vi "Measurement Logic.vi"() -> ()   [LabVIEW 2021, in "Crosstalk_PMIC.lvlib"]
uses:
  Crosstalk_PMIC.lvlib
  Measurement Configuration.ctl
  Measurement Results.ctl
  <vilib>/Plug-In SDKs/Measurements/Measure Call Context/Measure Call Context.lvclass
  <instrlib>/niDCPower/nidcpower.llb/niDCPower Sense.ctl
  <instrlib>/niDCPower/nidcpower.llb/niDCPower Source Mode.ctl
  <instrlib>/niDCPower/nidcpower.llb/niDCPower Wait For Event - Event.ctl
  <instrlib>/niDCPower/nidcpower.llb/niDCPower Measurement Type.ctl
  <instrlib>/niScope/Controls/niScope vertical coupling.ctl
  <instrlib>/niScope/Controls/niScope trigger slope.ctl
  <instrlib>/niScope/Controls/niScope trigger coupling.ctl
  <instrlib>/niScope/Controls/niScope trigger source.ctl
  <instrlib>/niDCPower/nidcpower.llb/niDCPower Get Channel Name From String.vi
  <instrlib>/niScope/Configure/Trigger/niScope Configure Trigger Edge.vi
  <instrlib>/niScope/Acquire/Fetch/niScope Multi Fetch WDT.vi
  <vilib>/Plug-In SDKs/Measurements/Measure Call Context/Accessor/Is Canceled.vi
panel:
  out "CrosstalkGraph":waveform(dbl)[](graph) caption="Ripple"
  out "measure call context out":refnum<class "Measure Call Context.lvclass">
  in  "measure call context in":refnum<class "Measure Call Context.lvclass">
  out "measurement results":T1
  in  "measurement configuration":T2={"Mode of operation"=enum."Perform measurement", "DUT setup time"=1.0, "Aperture time"=0.005, "Source resource name"="", "Source sense"=1009, "Source current limit"=25.0, "Source voltage level"=6.0, "Load resource name"="", "Load sense"=1009, "Load voltage limit range"=6.0, "Scope resource names"=[], "Scope channel names"=[], "Scope sample rate"=10000.0, "Scope acquisition time"=3.0, "Scope probe attenuation"=1.0, "Load current level"=0.005, "ExportData"=FALSE} {"Load sense" items=["Local"=1008, "Remote"=1009]; "Source sense" items=["Local"=1008, "Remote"=1009]}
  out "error out":errorcluster
  in  "error in":errorcluster
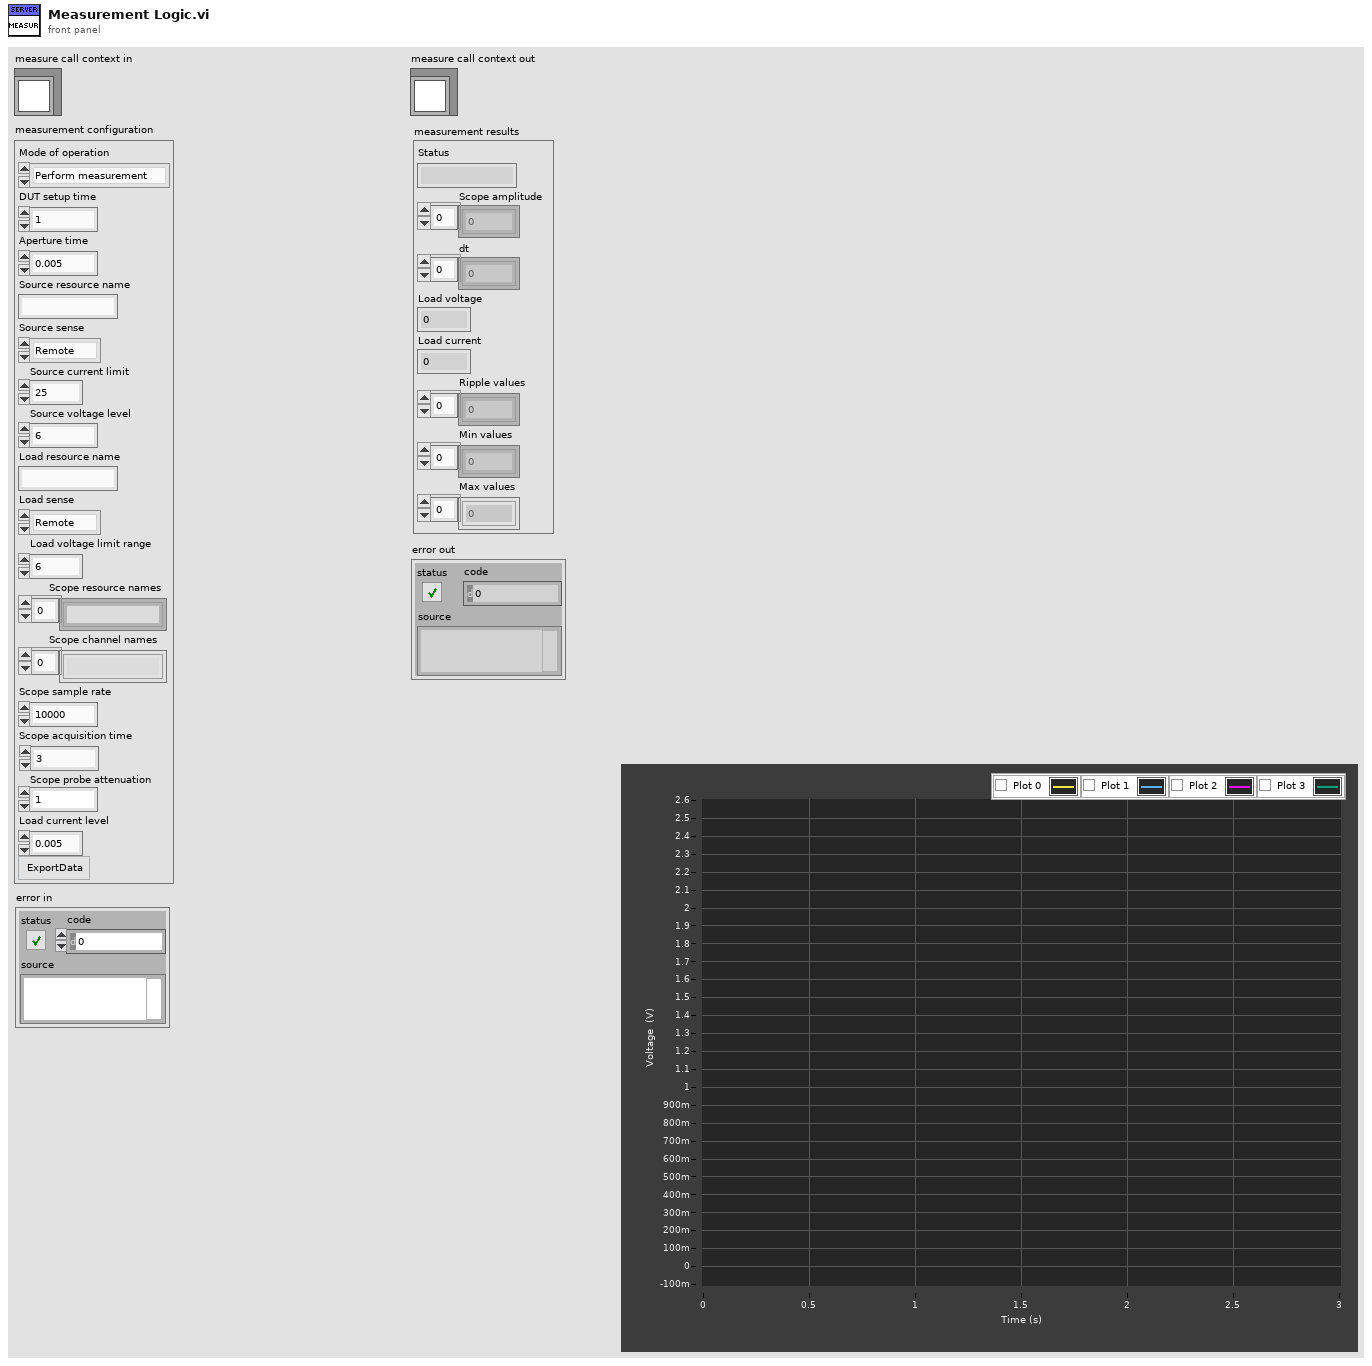
[diagram p1: front panel]
types:
  T1 = typedef "Crosstalk_PMIC.lvlib/Measurement Results.ctl" = cluster{"Status":string, "Scope amplitude":dbl[], "dt":dbl[], "Load voltage":dbl, "Load current":dbl, "Ripple values":dbl[], "Min values":dbl[], "Max values":dbl[]}
  T2 = typedef "Crosstalk_PMIC.lvlib/Measurement Configuration.ctl" = cluster{"Mode of operation":enum32{"Power on the DUT", "Perform measurement", "Power off the DUT"}, "DUT setup time":dbl, "Aperture time":dbl, "Source resource name":string, "Source sense":i32, "Source current limit":dbl, "Source voltage level":dbl, "Load resource name":string, "Load sense":i32, "Load voltage limit range":dbl, "Scope resource names":string[], "Scope channel names":string[], "Scope sample rate":dbl, "Scope acquisition time":dbl, "Scope probe attenuation":dbl, "Load current level":dbl, "ExportData":bool}
  T3 = cluster{"Source out":refnum<k15>, "Source channel name":string, "Load out":refnum<k15>, "Load channel name":string, "Scopes out":refnum<k15>[], "Scope channel names":string[], "Measurement Results":T1}
  T4 = enum32{"Power on the DUT", "Perform measurement", "Power off the DUT"}
  T5 = typedef "niScope trigger source.ctl" = string
  T6 = enum16{"open", "replace", "create", "open or create", "replace or create", "replace or create with confirmation"}
  T7 = typedef "niDCPower Wait For Event - Event.ctl" = i32
  T8 = typedef "niDCPower Source Mode.ctl" = i32
  T9 = typedef "niDCPower Sense.ctl" = i32
  T10 = typedef "niDCPower Measurement Type.ctl" = i32
  T11 = typedef "niScope vertical coupling.ctl" = i32
  T12 = typedef "niScope trigger coupling.ctl" = u16
  T13 = typedef "niScope trigger slope.ctl" = i32
  T14 = typedef "imagedata.ctl" = cluster{"image type":i32, "image depth":i32, "image":u8[], "mask":u8[], "colors":u32[], "Rectangle":cluster{"left":i16, "top":i16, "right":i16, "bottom":i16}}
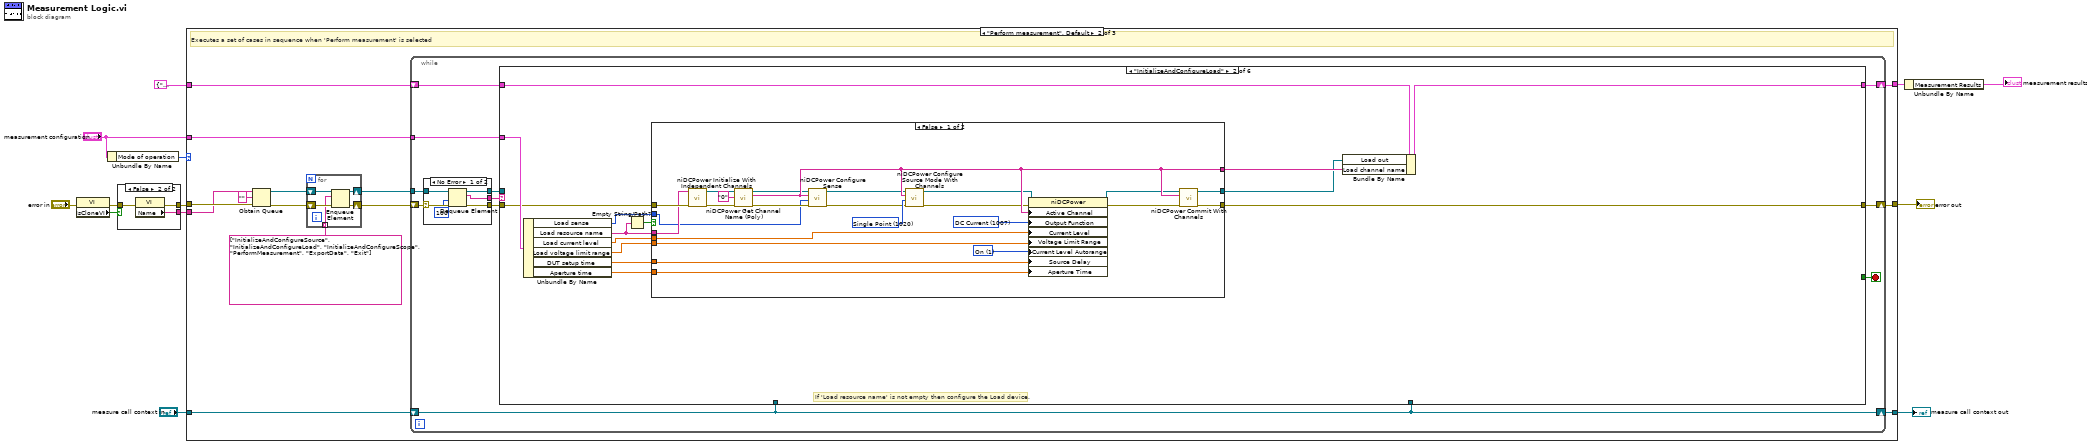
[diagram p0: block diagram]
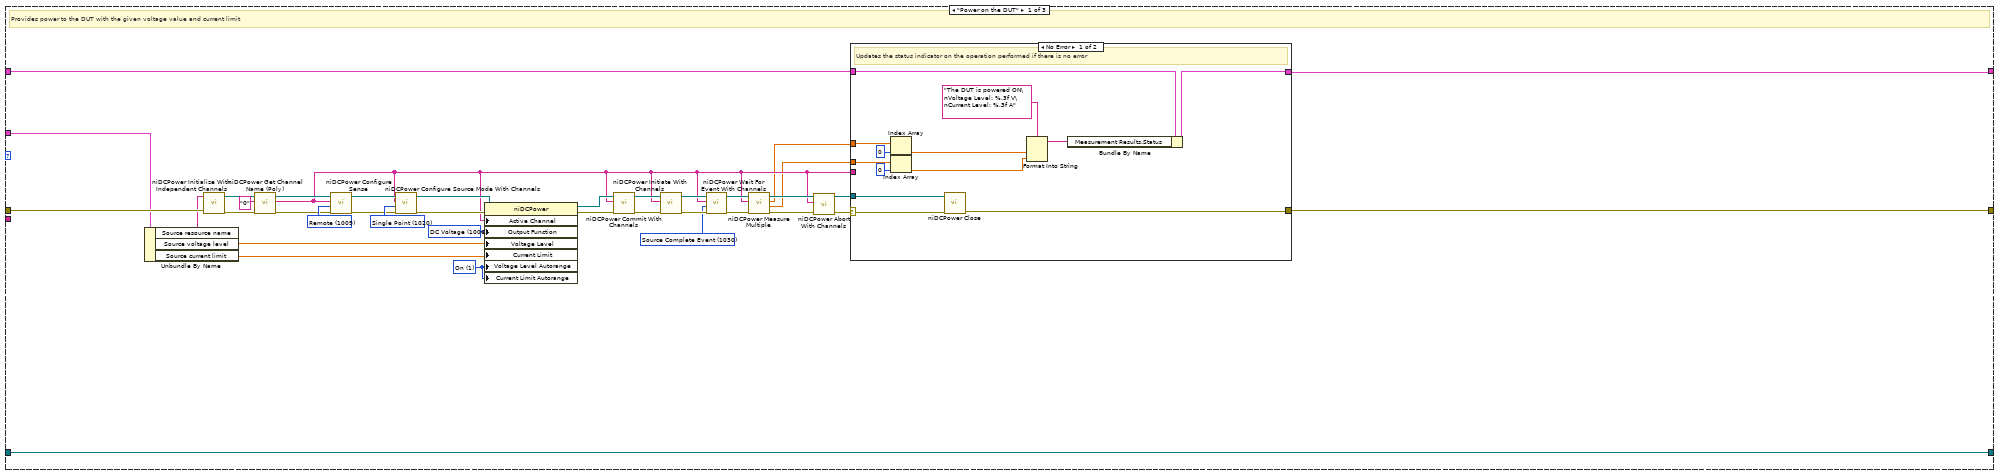
[diagram p2: hidden frame]
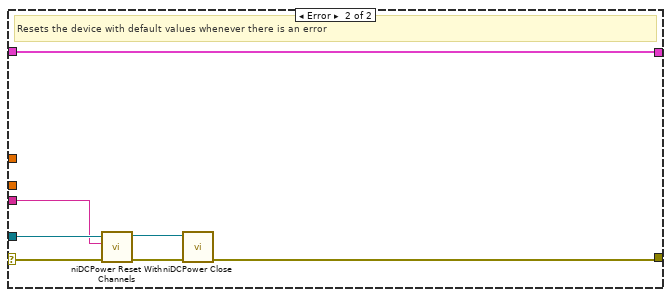
[diagram p3: hidden frame]
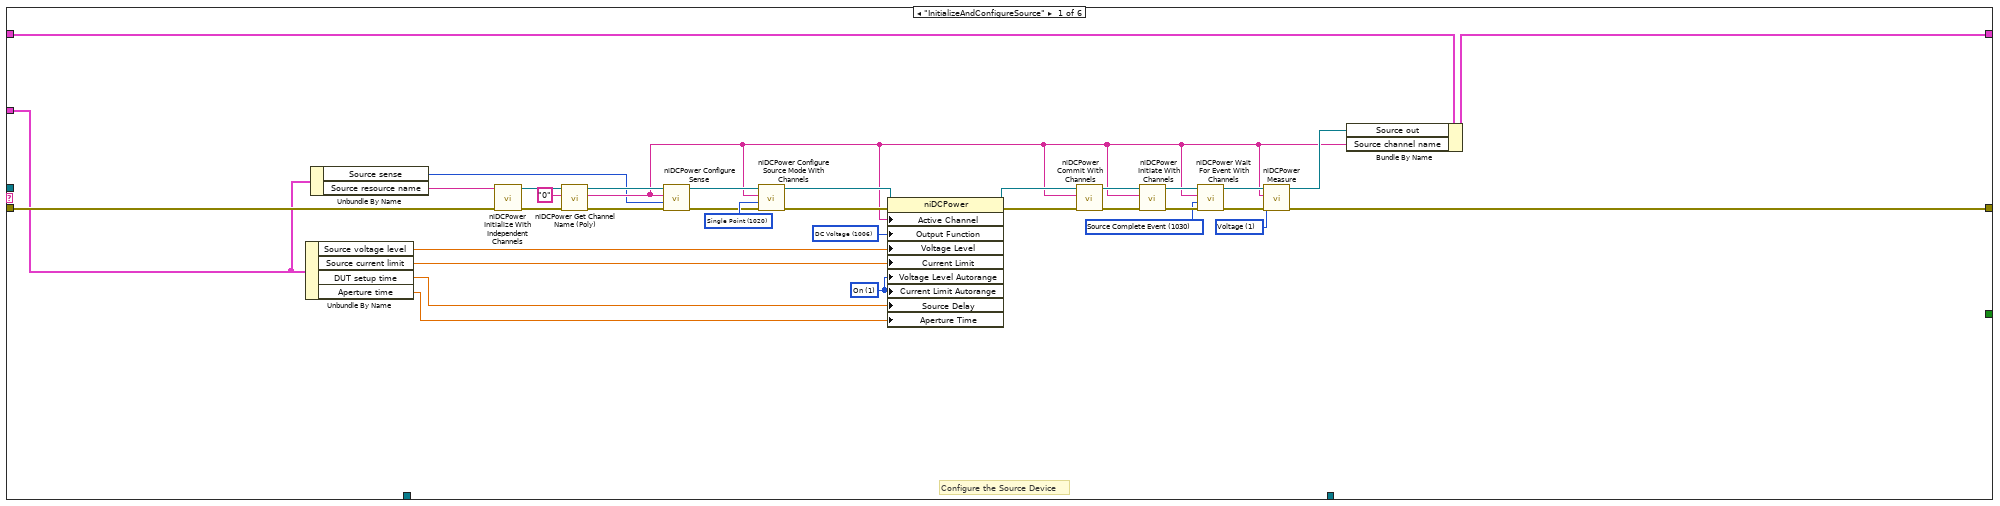
[diagram p4: hidden frame]
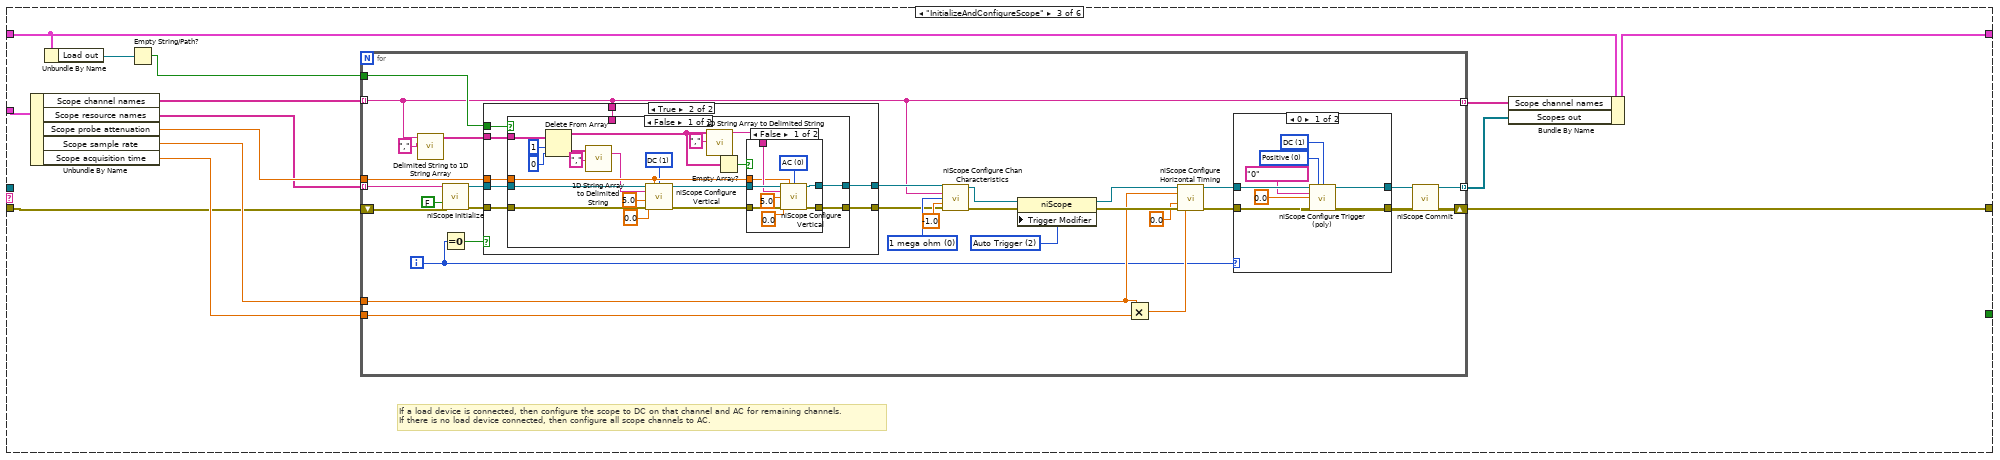
[diagram p6: hidden frame]
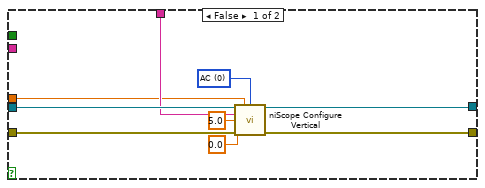
[diagram p7: hidden frame]
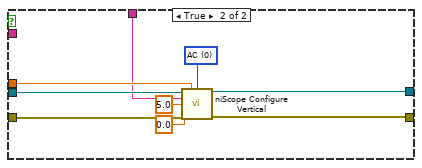
[diagram p9: hidden frame]
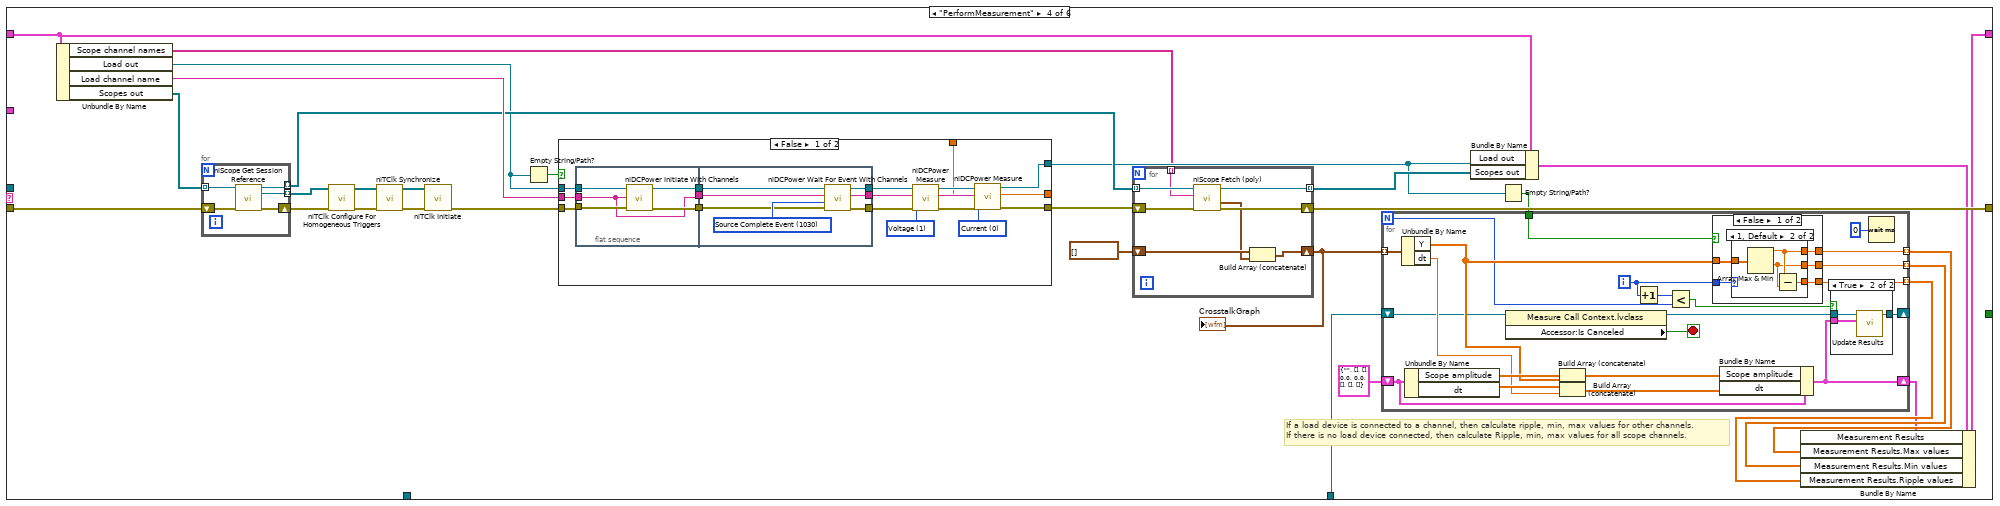
[diagram p11: hidden frame]
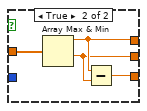
[diagram p15: hidden frame]
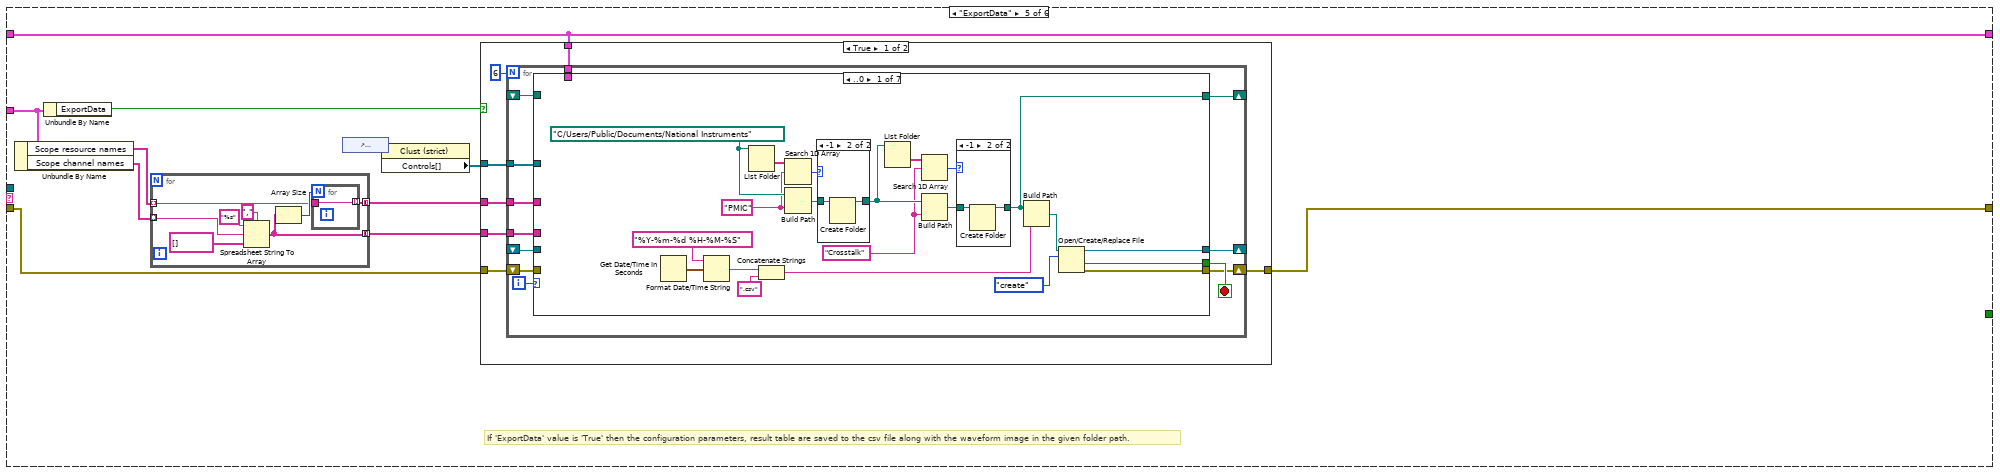
[diagram p16: hidden frame]
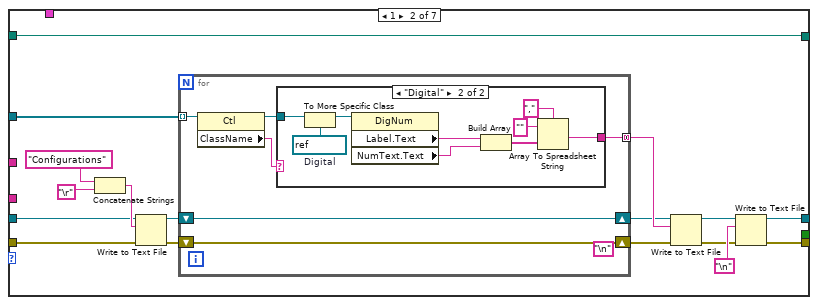
[diagram p19: hidden frame]
diagram:
  n1 = property class="VI"(error in="error in") -> (error out=w12:errorcluster, "IsCloneVI"=w13:bool)  [unwired: 1 in, 1 out]
  n2 = Unbundle By Name("measurement configuration") -> ("Mode of operation"=w7:T4)
  n3 = case shown="False" w13 {
    tunnel: [w16 w19] -> w10
    tunnel: [w15 w18] -> w9
    tunnel: w12 -> [w14 w17]
    frame True {
      n4 = property class="VI"(error in=w14) -> (error out=w16:errorcluster, "Clone Name"=w15:string)  [unwired: 1 in, 1 out]
    }
    frame False {
      n5 = property class="VI"(error in=w17) -> (error out=w19:errorcluster, "Name"=w18:string)  [unwired: 1 in, 1 out]
    }
  }
  n6 = case shown="\"Perform measurement\", Default" w7 {
    tunnel: [w21 w77 w667] -> w4
    tunnel: w10 -> [w37 w87 w666]
    tunnel: w9 -> [_ w86 _]
    tunnel: "measurement configuration" -> [w30 w83 w656]
    tunnel: [w22 w78 w653] -> w2
    tunnel: T3 {"Source out"="", "Source channel name"="", "Load out"="", "Load channel name"="", "Scopes out"=[], "Scope channel names"=[], "Measurement Results"={"Status"="", "Scope amplitude"=[], "dt"=[], "Load voltage"=0.0, "Load current"=0.0, "Ripple values"=[], "Min values"=[], "Max values"=[]}} -> [w23 w82 w654]
    tunnel: "measure call context in" -> [w20 w80 w655]
    tunnel: [w20 w79 w655] -> w5
    frame "Power on the DUT" {
      w40 = 1 items=["Off", "On"] ("Source:DC Voltage:Voltage Level Autorange")
      w41 = T7 1030 items=["Source Complete Event"=1030, "Measure Complete Event"=1031, "Sequence Iteration Complete Event"=1032, "Sequence Engine Done Event"=1033, "Pulse Complete Event"=1051, "Ready For Pulse Trigger Event"=1052] ("event")
      w52 = T8 1020 items=["Single Point"=1020, "Sequence"=1021] ("source mode")
      w47 = 1006 items=["DC Voltage"=1006, "DC Current"=1007, "Pulse Voltage"=1049, "Pulse Current"=1050] ("Source:Output Function")
      w42 = T9 1009 items=["Local"=1008, "Remote"=1009] ("sense")
      # "Provides power to the DUT with the given voltage value and current limit"
      n7 = Unbundle By Name(w30) -> ("Source resource name"=w34:string, "Source voltage level"=w29:dbl, "Source current limit"=w35:dbl)
      n8 = call <instrlib>:"niDCPower Initialize With Independent Channels.vi"("error in (no error)"=w37, "resource name"=w34) -> ("error out"=w39:errorcluster, "instrument handle out"=w43:refnum<k15>)  [unwired: 8 in]
      n9 = call-poly <instrlib>:"niDCPower Get Channel Name (Poly).vi"("index"="0", "instrument handle"=w43) -> ("name"=w26:string, "instrument handle out"=w38:refnum<k15>)  [unwired: 7 in, 1 out]
      n10 = call <instrlib>:"niDCPower Configure Sense.vi"("error in (no error)"=w39, "sense"=w42, "channel name"=w26, "instrument handle"=w38) -> ("error out"=w50:errorcluster, "instrument handle out"=w48:refnum<k15>)  [unwired: 6 in]
      n11 = call <instrlib>:"niDCPower Configure Source Mode With Channels.vi"("error in (no error)"=w50, "source mode"=w52, "channel name"=w26, "instrument handle"=w48) -> ("error out"=w51:errorcluster, "instrument handle out"=w49:refnum<k15>)  [unwired: 6 in]
      n12 = property class="niDCPower"(reference=w49, error in=w51, "Active Channel"=w26, "Output Function"=w47, "Voltage Level"=w29, "Current Limit"=w35, "Voltage Level Autorange"=w40, "Current Limit Autorange"=w40) -> (reference out=w53:refnum<k15>, error out=w54:errorcluster)
      n13 = call <instrlib>:"niDCPower Commit With Channels.vi"("error in (no error)"=w54, "channel name"=w26, "instrument handle"=w53) -> ("error out"=w56:errorcluster, "instrument handle out"=w55:refnum<k15>)  [unwired: 7 in]
      n14 = call <instrlib>:"niDCPower Initiate With Channels.vi"("error in (no error)"=w56, "channel name"=w26, "instrument handle"=w55) -> ("error out"=w44:errorcluster, "instrument handle out"=w45:refnum<k15>)  [unwired: 7 in]
      n15 = call <instrlib>:"niDCPower Wait For Event With Channels.vi"("error in (no error)"=w44, "event"=w41, "channel name"=w26, "instrument handle"=w45) -> ("error out"=w32:errorcluster, "instrument handle out"=w46:refnum<k15>)  [unwired: 6 in]
      n16 = call <instrlib>:"niDCPower Measure Multiple.vi"("error in (no error)"=w32, "channel name"=w26, "instrument handle"=w46) -> ("error out"=w31:errorcluster, "current measurements"=w24:dbl[], "voltage measurements"=w25:dbl[], "instrument handle out"=w33:refnum<k15>)  [unwired: 5 in]
      n17 = call <instrlib>:"niDCPower Abort With Channels.vi"("error in (no error)"=w31, "channel name"=w26, "instrument handle"=w33) -> ("error out"=w28:errorcluster, "instrument handle out"=w27:refnum<k15>)  [unwired: 7 in]
      n18 = case shown="No Error" w28 {
        selector: w28 -> [w69 w74]
        tunnel: [w68 w73] -> w21
        tunnel: [w67 w70] -> w22
        tunnel: w27 -> [w63 w72]
        tunnel: w26 -> [_ w71]
        tunnel: w25 -> [w62 _]
        tunnel: w24 -> [w61 _]
        tunnel: w23 -> [w60 w70]
        frame No Error {
          # "Updates the status indicator on the operation performed if there is no error"
          n19 = Index Array(array=w62, index=0) -> (element=w59:dbl)
          n20 = Index Array(array=w61, index=0) -> (element=w58:dbl)
          n21 = call <instrlib>:"niDCPower Close.vi"("error in (no error)"=w69, "instrument handle"=w63) -> ("error out"=w68:errorcluster)  [unwired: 9 out]
          n22 = Format Into String(format string="The DUT is powered ON\nVoltage Level: %.3f V\nCurrent Level: %.3f A" ("message"), w59, w58) -> (resulting string=w57:string)  [unwired: 2 in, 1 out]
          n23 = Bundle By Name(cluster=w60, "Measurement Results.Status"=w57) -> (w67:T3)
        }
        frame Error {
          # "Resets the device with default values whenever there is an error"
          n24 = call <instrlib>:"niDCPower Reset With Channels.vi"("error in (no error)"=w74, "channel name"=w71, "instrument handle"=w72) -> ("error out"=w76:errorcluster, "instrument handle out"=w75:refnum<k15>)  [unwired: 7 in]
          n25 = call <instrlib>:"niDCPower Close.vi"("error in (no error)"=w76, "instrument handle"=w75) -> ("error out"=w73:errorcluster)  [unwired: 9 out]
        }
      }
    }
    frame "Perform measurement", Default {
      # "Executes a set of cases in sequence when 'Perform measurement' is selected"
      n26 = Obtain Queue(name (unnamed)=w86, element data type="", error in (no error)=w87) -> (queue out=w89:refnum<queue>, error out=w90:errorcluster)  [unwired: 2 in, 1 out]
      n27 = for {
        shift-right: [w638] -> w84
        shift-left: w89 -> [w640]
        shift-right: [w637] -> w81
        shift-left: w90 -> [w639]
        tunnel: string[] ["InitializeAndConfigureSource", "InitializeAndConfigureLoad", "InitializeAndConfigureScope", "PerformMeasurement", "ExportData", "Exit"] ("Step sequence") -> [w636] mode=indexing
        n28 = Enqueue Element(queue=w640, element=w636, error in (no error)=w639) -> (queue out=w638:refnum<queue>, error out=w637:errorcluster)  [unwired: 1 in, 1 out]
      }
      n29 = while {
        tunnel: w84 -> [w101]
        tunnel: w83 -> [w98]
        shift-right: [w95] -> w78
        shift-left: w82 -> [w96]
        shift-right: [w94] -> w77
        shift-left: w81 -> [w100]
        shift-right: [w91] -> w79
        shift-left: w80 -> [w91]
        stop <- w93 stop-if-true
        n30 = case shown="No Error" w100 {
          selector: w100 -> [w630 w634]
          tunnel: w101 -> [w632 w633]
          tunnel: [w631 "Exit" ("t")] -> w92
          tunnel: [w629 w634] -> w97
          tunnel: [w627 w633] -> w99
          frame No Error {
            n31 = Dequeue Element(queue=w632, timeout in ms (-1)=100, error in (no error)=w630) -> (queue out=w627:refnum<queue>, element=w631:string, error out=w629:errorcluster)  [unwired: 1 out]
          }
          frame Error {
          }
        }
        n32 = case shown="\"InitializeAndConfigureLoad\"" w92 {
          tunnel: w99 -> [_ _ _ _ _ w569]
          tunnel: w98 -> [w112 w150 w189 _ w406 _]
          tunnel: w97 -> [w114 w149 w183 w306 w408 w574]
          tunnel: w96 -> [w133 w145 w178 w316 w400 w572]
          tunnel: [w134 w147 w184 w310 w400 w570] -> w95
          tunnel: [w136 w148 w182 w314 w407 w571] -> w94
          tunnel: w91 -> [_ _ _ _ _ _]
          tunnel: [_ _ _ _ _ TRUE] -> w93
          tunnel: w91 -> [_ _ _ w289 _ _]
          frame "InitializeAndConfigureSource" {
            w103 = T10 1 items=["Current", "Voltage"] ("measurement type")
            w116 = 1 items=["Off", "On"] ("Source:DC Voltage:Voltage Level Autorange")
            w117 = T7 1030 items=["Source Complete Event"=1030, "Measure Complete Event"=1031, "Sequence Iteration Complete Event"=1032, "Sequence Engine Done Event"=1033, "Pulse Complete Event"=1051, "Ready For Pulse Trigger Event"=1052] ("event")
            w128 = T8 1020 items=["Single Point"=1020, "Sequence"=1021] ("source mode")
            w123 = 1006 items=["DC Voltage"=1006, "DC Current"=1007, "Pulse Voltage"=1049, "Pulse Current"=1050] ("Source:Output Function")
            # "Configure the Source Device"
            n33 = Unbundle By Name(w112) -> ("Source voltage level"=w105:dbl, "Source current limit"=w113:dbl, "DUT setup time"=w115:dbl, "Aperture time"=w104:dbl)
            n34 = Unbundle By Name(w112) -> ("Source sense"=w102:i32, "Source resource name"=w111:string)
            n35 = call <instrlib>:"niDCPower Initialize With Independent Channels.vi"("error in (no error)"=w114, "resource name"=w111) -> ("error out"=w107:errorcluster, "instrument handle out"=w118:refnum<k15>)  [unwired: 8 in]
            n36 = call-poly <instrlib>:"niDCPower Get Channel Name (Poly).vi"("error in (no error)"=w107, "index"="0", "instrument handle"=w118) -> ("error out"=w106:errorcluster, "name"=w108:string, "instrument handle out"=w110:refnum<k15>)  [unwired: 6 in]
            n37 = call <instrlib>:"niDCPower Configure Sense.vi"("error in (no error)"=w106, "sense"=w102, "channel name"=w108, "instrument handle"=w110) -> ("error out"=w126:errorcluster, "instrument handle out"=w124:refnum<k15>)  [unwired: 6 in]
            n38 = call <instrlib>:"niDCPower Configure Source Mode With Channels.vi"("error in (no error)"=w126, "source mode"=w128, "channel name"=w108, "instrument handle"=w124) -> ("error out"=w127:errorcluster, "instrument handle out"=w125:refnum<k15>)  [unwired: 6 in]
            n39 = property class="niDCPower"(reference=w125, error in=w127, "Active Channel"=w108, "Output Function"=w123, "Voltage Level"=w105, "Current Limit"=w113, "Voltage Level Autorange"=w116, "Current Limit Autorange"=w116, "Source Delay"=w115, "Aperture Time"=w104) -> (reference out=w129:refnum<k15>, error out=w130:errorcluster)
            n40 = call <instrlib>:"niDCPower Commit With Channels.vi"("error in (no error)"=w130, "channel name"=w108, "instrument handle"=w129) -> ("error out"=w132:errorcluster, "instrument handle out"=w131:refnum<k15>)  [unwired: 7 in]
            n41 = call <instrlib>:"niDCPower Initiate With Channels.vi"("error in (no error)"=w132, "channel name"=w108, "instrument handle"=w131) -> ("error out"=w119:errorcluster, "instrument handle out"=w120:refnum<k15>)  [unwired: 7 in]
            n42 = call <instrlib>:"niDCPower Wait For Event With Channels.vi"("error in (no error)"=w119, "event"=w117, "channel name"=w108, "instrument handle"=w120) -> ("error out"=w122:errorcluster, "instrument handle out"=w121:refnum<k15>)  [unwired: 6 in]
            n43 = call <instrlib>:"niDCPower Measure.vi"("error in (no error)"=w122, "measurement type"=w103, "channel name"=w108, "instrument handle"=w121) -> ("error out"=w136:errorcluster, "instrument handle out"=w135:refnum<k15>)  [unwired: 5 in, 1 out]
            n44 = Bundle By Name(cluster=w133, "Source out"=w135, "Source channel name"=w108) -> (w134:T3)
          }
          frame "InitializeAndConfigureLoad" {
            # "If 'Load resource name' is not empty then configure the Load device."
            n45 = Unbundle By Name(w150) -> ("Load sense"=w137:i32, "Load resource name"=w139:string, "Load current level"=w141:dbl, "Load voltage limit range"=w142:dbl, "DUT setup time"=w146:dbl, "Aperture time"=w140:dbl)
            n46 = Empty String/Path?(string/path=w139) -> (empty?=w138:bool)
            n47 = case shown="False" w138 {
              tunnel: w149 -> [w174 w175]
              tunnel: [w173 w175] -> w148
              tunnel: w146 -> [w172 _]
              tunnel: [w171 _] -> w144
              tunnel: [w170 _] -> w143
              tunnel: w142 -> [w169 _]
              tunnel: w141 -> [w168 _]
              tunnel: w140 -> [w167 _]
              tunnel: w139 -> [w152 _]
              tunnel: w137 -> [w151 _]
              frame False {
                w164 = T8 1020 items=["Single Point"=1020, "Sequence"=1021] ("source mode")
                w157 = 1 items=["Off", "On"] ("Source:DC Current:Current Level Autorange")
                w158 = 1007 items=["DC Voltage"=1006, "DC Current"=1007, "Pulse Voltage"=1049, "Pulse Current"=1050] ("Source:Output Function")
                n48 = call <instrlib>:"niDCPower Initialize With Independent Channels.vi"("error in (no error)"=w174, "resource name"=w152) -> ("error out"=w154:errorcluster, "instrument handle out"=w159:refnum<k15>)  [unwired: 8 in]
                n49 = call-poly <instrlib>:"niDCPower Get Channel Name (Poly).vi"("error in (no error)"=w154, "index"="0", "instrument handle"=w159) -> ("error out"=w153:errorcluster, "name"=w171:string, "instrument handle out"=w156:refnum<k15>)  [unwired: 6 in]
                n50 = call <instrlib>:"niDCPower Configure Sense.vi"("error in (no error)"=w153, "sense"=w151, "channel name"=w171, "instrument handle"=w156) -> ("error out"=w161:errorcluster, "instrument handle out"=w160:refnum<k15>)  [unwired: 6 in]
                n51 = call <instrlib>:"niDCPower Configure Source Mode With Channels.vi"("error in (no error)"=w161, "source mode"=w164, "channel name"=w171, "instrument handle"=w160) -> ("error out"=w163:errorcluster, "instrument handle out"=w162:refnum<k15>)  [unwired: 6 in]
                n52 = property class="niDCPower"(reference=w162, error in=w163, "Active Channel"=w171, "Output Function"=w158, "Current Level"=w168, "Voltage Limit Range"=w169, "Current Level Autorange"=w157, "Source Delay"=w172, "Aperture Time"=w167) -> (reference out=w165:refnum<k15>, error out=w166:errorcluster)
                n53 = call <instrlib>:"niDCPower Commit With Channels.vi"("error in (no error)"=w166, "channel name"=w171, "instrument handle"=w165) -> ("error out"=w173:errorcluster, "instrument handle out"=w170:refnum<k15>)  [unwired: 7 in]
              }
              frame True {
              }
            }
            n54 = Bundle By Name(cluster=w145, "Load out"=w143, "Load channel name"=w144) -> (w147:T3)
          }
          frame "InitializeAndConfigureScope" {
            # "If a load device is connected, then configure the scope to DC on that channel and AC for remaining channels.\nIf there is no load device connected, then configure all scope channels to AC."
            n55 = Unbundle By Name(w189) -> ("Scope channel names"=w179:string[], "Scope resource names"=w180:string[], "Scope probe attenuation"=w188:dbl, "Scope sample rate"=w187:dbl, "Scope acquisition time"=w186:dbl)
            n56 = Unbundle By Name(w178) -> ("Load out"=w177:refnum<k15>)
            n57 = Empty String/Path?(string/path=w177) -> (empty?=w176:bool)
            n58 = for {
              tunnel: w180 -> [w207] mode=indexing
              tunnel: w179 -> [w192] mode=indexing
              tunnel: [w205] -> w185 mode=indexing
              tunnel: w188 -> [w194]
              tunnel: w187 -> [w204]
              tunnel: w186 -> [w203]
              shift-right: [w201] -> w182
              shift-left: w183 -> [w202]
              tunnel: [w192] -> w181 mode=indexing
              tunnel: w176 -> [w193]
              i -> [w191]
              w215 = 2 items=["None"=1, "Auto Trigger"=2] ("Triggering:Trigger Modifier")
              w219 = u32 0 items=["1 mega ohm"=0, "50 ohms"=2] ("input impedance")
              n59 = call <vilib>:"Delimited String to 1D String Array.vi"("delimiter"=",", "delimited string"=w192) -> ("string array"=w199:string[])  [unwired: 9 in]
              n60 = call <instrlib>:"niScope Initialize.vi"("resource name"=w207, "reset device"=FALSE, "error in"=w202) -> ("instrument handle"=w197:refnum<k15>, "error out"=w196:errorcluster)  [unwired: 11 in]
              n61 = Equal To 0?(x=w191) -> (x = 0?=w190:bool)
              n62 = case shown="True" w190 {
                tunnel: w199 -> [_ w237]
                tunnel: [w228 w236] -> w198
                tunnel: w197 -> [w229 w235]
                tunnel: w196 -> [w227 w234]
                tunnel: [w226 w233] -> w195
                tunnel: w194 -> [w221 w232]
                tunnel: w193 -> [_ w231]
                tunnel: w192 -> [w225 w230]
                frame False {
                  w224 = T11 0 items=["AC", "DC", "Ground"] ("vertical coupling")
                  n63 = call <instrlib>:"niScope Configure Vertical.vi"("instrument handle"=w229, "probe attenuation"=w221, "vertical coupling"=w224, "channels"=w225, "vertical range"=5.0, "vertical offset"=0.0, "error in"=w227) -> ("instrument handle out"=w228:refnum<k15>, "error out"=w226:errorcluster)  [unwired: 7 in]
                }
                frame True {
                  n64 = case shown="False" w231 {
                    tunnel: w237 -> [w257 _]
                    tunnel: [w253 w276] -> w236
                    tunnel: w235 -> [w252 w277]
                    tunnel: w234 -> [w251 w275]
                    tunnel: [w250 w274] -> w233
                    tunnel: w232 -> [w248 w270]
                    tunnel: w230 -> [_ w269]
                    frame False {
                      w243 = T11 1 items=["AC", "DC", "Ground"] ("vertical coupling")
                      n65 = Delete From Array(array=w257, length=1, index=0) -> (deleted portion=w246:string[], array with subset deleted=w238:string[])
                      n66 = call <vilib>:"1D String Array to Delimited String.vi"("delimiter"=",", "string array"=w246) -> ("delimited string"=w247:string)  [unwired: 9 in]
                      n67 = call <instrlib>:"niScope Configure Vertical.vi"("instrument handle"=w252, "probe attenuation"=w248, "vertical coupling"=w243, "channels"=w247, "vertical range"=5.0, "vertical offset"=0.0, "error in"=w251) -> ("instrument handle out"=w254:refnum<k15>, "error out"=w249:errorcluster)  [unwired: 7 in]
                      n68 = call <vilib>:"1D String Array to Delimited String.vi"("delimiter"=",", "string array"=w238) -> ("delimited string"=w239:string)  [unwired: 9 in]
                      n69 = Empty Array?(array=w238) -> (empty?=w240:bool)
                      n70 = case shown="False" w240 {
                        tunnel: w254 -> [w266 w268]
                        tunnel: w239 -> [w265 _]
                        tunnel: [w264 w268] -> w253
                        tunnel: [w263 w267] -> w250
                        tunnel: w249 -> [w262 w267]
                        tunnel: w248 -> [w258 _]
                        frame False {
                          w260 = T11 0 items=["AC", "DC", "Ground"] ("vertical coupling")
                          n71 = call <instrlib>:"niScope Configure Vertical.vi"("instrument handle"=w266, "probe attenuation"=w258, "vertical coupling"=w260, "channels"=w265, "vertical range"=5.0, "vertical offset"=0.0, "error in"=w262) -> ("instrument handle out"=w264:refnum<k15>, "error out"=w263:errorcluster)  [unwired: 7 in]
                        }
                        frame True {
                        }
                      }
                    }
                    frame True {
                      w271 = T11 0 items=["AC", "DC", "Ground"] ("vertical coupling")
                      n72 = call <instrlib>:"niScope Configure Vertical.vi"("instrument handle"=w277, "probe attenuation"=w270, "vertical coupling"=w271, "channels"=w269, "vertical range"=5.0, "vertical offset"=0.0, "error in"=w275) -> ("instrument handle out"=w276:refnum<k15>, "error out"=w274:errorcluster)  [unwired: 7 in]
                    }
                  }
                }
              }
              n73 = call <instrlib>:"niScope Configure Chan Characteristics.vi"("instrument handle"=w198, "channels"=w192, "input impedance"=w219, "maximum input frequency"=-1.0, "error in"=w195) -> ("instrument handle out"=w217:refnum<k15>, "error out"=w216:errorcluster)  [unwired: 9 in]
              n74 = property class="niScope"(reference=w217, error in=w216, "Trigger Modifier"=w215) -> (reference out=w214:refnum<k15>, error out=w213:errorcluster)
              n75 = Multiply(x=w204, y=w203) -> (x*y=w208:dbl)
              n76 = call <instrlib>:"niScope Configure Horizontal Timing.vi"("instrument handle"=w214, "min sample rate"=w204, "reference position"=0.0, "error in"=w213, "min record length"=w208) -> ("instrument handle out"=w212:refnum<k15>, "error out"=w211:errorcluster)  [unwired: 9 in]
              n77 = case shown="0" w191 {
                tunnel: w212 -> [w284 w287]
                tunnel: w211 -> [w283 w286]
                tunnel: [w281 w286] -> w209
                tunnel: [w282 w287] -> w206
                frame 0 {
                  w285 = T12 1 items=["AC"=0, "DC"=1, "HF Reject"=3, "LF Reject"=4, "AC Plus HF Reject"=1001] ("trigger coupling")
                  w280 = T13 0 items=["Positive", "Negative"] ("trigger slope")
                  n78 = call-poly <instrlib>:"niScope Configure Trigger (poly).vi"("instrument handle"=w284, "trigger slope"=w280, "trigger coupling"=w285, "trigger source"=T5 "0", "trigger level"=0.0, "error in"=w283) -> ("instrument handle out"=w282:refnum<k15>, "error out"=w281:errorcluster)  [unwired: 8 in]
                }
                frame 1, Default {
                }
              }
              n79 = call <instrlib>:"niScope Commit.vi"("instrument handle"=w206, "error in"=w209) -> ("instrument handle out"=w205:refnum<k15>, "error out"=w201:errorcluster)  [unwired: 12 in]
            }
            n80 = Bundle By Name(cluster=w178, "Scope channel names"=w181, "Scopes out"=w185) -> (w184:T3)
          }
          frame "PerformMeasurement" {
            # "If a load device is connected to a channel, then calculate ripple, min, max values for other channels.\nIf there is no load device connected, then calculate Ripple, min, max values for all scope channels."
            n81 = Unbundle By Name(w316) -> ("Scope channel names"=w292:string[], "Load out"=w305:refnum<k15>, "Load channel name"=w317:string, "Scopes out"=w307:refnum<k15>[])
            n82 = for {
              tunnel: [w320] -> w299 mode=indexing
              shift-right: [w321] -> w298
              shift-left: w306 -> [w322]
              tunnel: [w319] -> w309 mode=indexing
              tunnel: w307 -> [w318] mode=indexing
              n83 = call <instrlib>:"niScope Get Session Reference.vi"("instrument handle"=w318, "error in"=w322) -> ("instrument handle out"=w319:refnum<k15>, "session reference"=w320:refnum<k20>, "error out"=w321:errorcluster)  [unwired: 11 in]
            }
            n84 = call <instrlib>:"niTClk Configure For Homogeneous Triggers.vi"("error in (no error)"=w298, "sessions"=w299) -> ("error out"=w300:errorcluster, "sessions out"=w301:refnum<k20>[])  [unwired: 8 in]
            n85 = call <instrlib>:"niTClk Synchronize.vi"("error in (no error)"=w300, "sessions"=w301) -> ("error out"=w302:errorcluster, "sessions out"=w303:refnum<k20>[])  [unwired: 8 in]
            n86 = call <instrlib>:"niTClk Initiate.vi"("error in (no error)"=w302, "sessions"=w303) -> ("error out"=w308:errorcluster)  [unwired: 8 in, 1 out]
            n87 = Empty String/Path?(string/path=w305) -> (empty?=w304:bool)
            n88 = case shown="False" w304 {
              tunnel: w317 -> [w336 _]
              tunnel: [w335 w352] -> w297
              tunnel: [w334 w351] -> w315
              tunnel: w308 -> [w333 w351]
              tunnel: w305 -> [w325 w352]
              tunnel: [w324 _] -> _
              tunnel: [w323 _] -> _
              frame False {
                w326 = T10 0 items=["Current", "Voltage"] ("measurement type")
                w328 = T10 1 items=["Current", "Voltage"] ("measurement type")
                n89 = flat-sequence {
                  tunnel: [w344] -> w339
                  tunnel: [w343] -> w338
                  tunnel: w333 -> [w342]
                  tunnel: w325 -> [w340]
                  tunnel: [w341] -> w337
                  tunnel: w336 -> [w341]
                  tunnel: w339 -> [w349]
                  tunnel: w338 -> [w346]
                  tunnel: [w347] -> w331
                  tunnel: [w348] -> w332
                  tunnel: w337 -> [w345]
                  tunnel: [w345] -> w327
                  frame #0 {
                    n90 = call <instrlib>:"niDCPower Initiate With Channels.vi"("error in (no error)"=w342, "channel name"=w341, "instrument handle"=w340) -> ("error out"=w344:errorcluster, "instrument handle out"=w343:refnum<k15>)  [unwired: 7 in]
                  }
                  frame #1 {
                    w350 = T7 1030 items=["Source Complete Event"=1030, "Measure Complete Event"=1031, "Sequence Iteration Complete Event"=1032, "Sequence Engine Done Event"=1033] ("event")
                    n91 = call <instrlib>:"niDCPower Wait For Event With Channels.vi"("error in (no error)"=w349, "event"=w350, "channel name"=w345, "instrument handle"=w346) -> ("error out"=w347:errorcluster, "instrument handle out"=w348:refnum<k15>)  [unwired: 6 in]
                  }
                }
                n92 = call <instrlib>:"niDCPower Measure.vi"("error in (no error)"=w331, "measurement type"=w328, "channel name"=w327, "instrument handle"=w332) -> ("error out"=w329:errorcluster, "measurement"=w324:dbl, "instrument handle out"=w330:refnum<k15>)  [unwired: 5 in]
                n93 = call <instrlib>:"niDCPower Measure.vi"("error in (no error)"=w329, "measurement type"=w326, "channel name"=w327, "instrument handle"=w330) -> ("error out"=w334:errorcluster, "measurement"=w323:dbl, "instrument handle out"=w335:refnum<k15>)  [unwired: 5 in]
              }
              frame True {
              }
            }
            n94 = for {
              shift-right: [w398] -> w314
              shift-left: w315 -> [w399]
              tunnel: w309 -> [w397] mode=indexing
              shift-right: [w395] -> w291
              shift-left: waveform(dbl)[] [] -> [w396]
              tunnel: [w394] -> w313 mode=indexing
              tunnel: w292 -> [w393] mode=indexing
              n95 = call-poly <instrlib>:"niScope Fetch (poly).vi"("error in"=w399, "channels"=w393, "instrument handle"=w397) -> ("error out"=w398:errorcluster, "wfm"=w392:waveform(dbl)[], "instrument handle out"=w394:refnum<k15>)  [unwired: 5 in, 1 out]
              n96 = Build Array (concatenate)(w396, w392) -> (w395:waveform(dbl)[])
            }
            "CrosstalkGraph" <- w291
            n97 = Bundle By Name(cluster=w316, "Load out"=w297, "Scopes out"=w313) -> (w311:T3)
            n98 = Empty String/Path?(string/path=w297) -> (empty?=w296:bool)
            n99 = for {
              N -> [w358]
              tunnel: w291 -> [w374] mode=indexing
              tunnel: [w373] -> w295 mode=indexing
              tunnel: [w372] -> w294 mode=indexing
              tunnel: w296 -> [w371]
              tunnel: [w370] -> w293 mode=indexing
              shift-right: [w356] -> w288
              shift-left: T1 {"Status"="", "Scope amplitude"=[], "dt"=[], "Load voltage"=0.0, "Load current"=0.0, "Ripple values"=[], "Min values"=[], "Max values"=[]} ("Measurement Results") -> [w365]
              shift-right: [w354] -> _
              shift-left: w289 -> [w362]
              i -> [w359]
              stop <- w361 stop-if-true
              n100 = Unbundle By Name(w374) -> ("Y"=w368:dbl[], "dt"=w366:dbl)
              n101 = Unbundle By Name(w365) -> ("Scope amplitude"=w369:dbl[], "dt"=w367:dbl[])
              n102 = property class="Measure Call Context.lvclass"(reference=w362) -> (reference out=w355:refnum<class "Measure Call Context.lvclass">, "Accessor:Is Canceled"=w361:bool)  [unwired: 1 in, 1 out]
              n103 = Build Array (concatenate)(w369, w368) -> (w364:dbl[])
              n104 = Build Array (concatenate)(w367, w366) -> (w363:dbl[])
              n105 = Increment(x=w359) -> (x+1=w360:i32)
              n106 = Less?(x=w360, y=w358) -> (x < y?=w357:bool)
              n107 = case shown="False" w371 {
                tunnel: w368 -> [w382 w391]
                tunnel: [w381 w389] -> w373
                tunnel: [w380 w388] -> w372
                tunnel: w359 -> [w383 _]
                tunnel: [w379 w390] -> w370
                frame False {
                  n108 = case shown="1, Default" w383 {
                    tunnel: w382 -> [_ w387]
                    tunnel: [_ w386] -> w381
                    tunnel: [_ w385] -> w380
                    tunnel: [_ w384] -> w379
                    frame 0 {
                    }
                    frame 1, Default {
                      n109 = Array Max & Min(array=w387) -> (max value=w386:dbl, min value=w385:dbl)  [unwired: 2 out]
                      n110 = Subtract(x=w386, y=w385) -> (x-y=w384:dbl)
                    }
                  }
                }
                frame True {
                  n111 = Array Max & Min(array=w391) -> (max value=w389:dbl, min value=w388:dbl)  [unwired: 2 out]
                  n112 = Subtract(x=w389, y=w388) -> (x-y=w390:dbl)
                }
              }
              n113 = Bundle By Name(cluster=w365, "Scope amplitude"=w364, "dt"=w363) -> (w356:T1)
              n114 = case shown="True" w357 {
                tunnel: [w375 w378] -> w354
                tunnel: w356 -> [_ w377]
                tunnel: w355 -> [w375 w376]
                frame False {
                }
                frame True {
                  n115 = call <vilib>:"Update Results.vi"("measurement results"=w377, "measure call context in"=w376) -> ("measure call context out"=w378:refnum<class "Measure Call Context.lvclass">)  [unwired: 8 in, 1 out]
                }
              }
              n116 = Wait (ms)(milliseconds to wait=u32 0) -> ()  [unwired: 1 out]
            }
            n117 = Bundle By Name(cluster=w311, "Measurement Results"=w288, "Measurement Results.Max values"=w295, "Measurement Results.Min values"=w294, "Measurement Results.Ripple values"=w293) -> (w310:T3)
          }
          frame "ExportData" {
            # "If 'ExportData' value is 'True' then the configuration parameters, result table are saved to the csv file along with the waveform image in the given folder path."
            n118 = Unbundle By Name(w406) -> ("Scope resource names"=w405:string[], "Scope channel names"=w404:string[])
            n119 = Unbundle By Name(w406) -> ("ExportData"=w409:bool)
            n120 = for {
              tunnel: [w415] -> w401 mode=concatenating
              tunnel: [w413] -> w402 mode=concatenating
              tunnel: w405 -> [w412] mode=indexing
              tunnel: w404 -> [w411] mode=indexing
              n121 = Spreadsheet String To Array(delimiter (Tab)=",", format string="%s", spreadsheet string=w411, array type (2D Dbl)=string[] []) -> (array=w415:string[])
              n122 = Array Size(array=w415) -> (size(s)=w414:i32)
              n123 = for {
                N: w414 -> [_]
                tunnel: w412 -> [w419]
                tunnel: [w419] -> w413 mode=indexing
              }
            }
            n124 = control-ref of="measurement configuration"() -> (w410:refnum<vi>)
            n125 = property class="Clust (strict)"(reference=w410) -> ("Controls[]"=w403:refnum<vi>[])  [unwired: 1 in, 2 out]
            n126 = case shown="True" w409 {
              tunnel: w403 -> [w425 _]
              tunnel: w408 -> [w424 w567]
              tunnel: [w423 w567] -> w407
              tunnel: w402 -> [w422 _]
              tunnel: w401 -> [w421 _]
              tunnel: w400 -> [w420 _]
              frame True {
                n127 = for {
                  N: 6 -> [_]
                  shift-right: [w436] -> _
                  shift-left: _ -> [w435]
                  shift-right: [w434] -> w423
                  shift-left: w424 -> [w433]
                  tunnel: w425 -> [w432]
                  tunnel: w422 -> [w431]
                  tunnel: w421 -> [w430]
                  tunnel: w420 -> [w429]
                  shift-right: [w428] -> _
                  shift-left: _ -> [w427]
                  i -> [w438]
                  stop <- w437 stop-if-true
                  n128 = case shown="..0" w438 {
                    tunnel: [w452 _ _ _ _ _ _] -> w437
                    tunnel: [w458 w467 w505 w525 refnum<file> refnum ("refnum out") w562 w566] -> w436
                    tunnel: w435 -> [_ w478 w514 w532 w553 w562 w566]
                    tunnel: [w451 w469 w504 w524 w551 w563 w565] -> w434
                    tunnel: w433 -> [_ w476 w513 w531 w550 w563 w565]
                    tunnel: w432 -> [_ w479 _ _ _ _ _]
                    tunnel: w431 -> [_ _ _ w522 _ _ _]
                    tunnel: w430 -> [_ _ _ w521 _ _ _]
                    tunnel: w429 -> [_ _ _ w520 _ _ _]
                    tunnel: [w439 w466 w498 w515 w549 w556 w564] -> w428
                    tunnel: w427 -> [_ w466 w498 w515 w549 w556 w564]
                    frame ..0 {
                      w447 = "Crosstalk" ("prompt")
                      w454 = "PMIC" ("prompt")
                      w457 = path "C:/Users/Public/Documents/National Instruments" ("base path")
                      n129 = Get Date/Time In Seconds() -> (seconds since 1Jan1904=w444:timestamp)
                      n130 = Format Date/Time String(time format string (%c)="%Y-%m-%d %H-%M-%S", seconds (now)=w444) -> (date/time string=w443:string)  [unwired: 1 in]
                      n131 = List Folder(path=w457) -> (folder names=w455:string[])  [unwired: 3 in, 3 out]
                      n132 = Concatenate Strings(w443, ".csv" ("string")) -> (w441:string)
                      n133 = Search 1D Array(1D array=w455, element=w454) -> (index of element=w453:i32)  [unwired: 1 in]
                      n134 = Build Path(base path=w457, name or relative path=w454) -> (appended path=w456:path)
                      n135 = case shown="-1" w453 {
                        tunnel: w456 -> [w463 w465]
                        tunnel: [w463 w464] -> w448
                        frame Default {
                        }
                        frame -1 {
                          n136 = Create Folder(path (use dialog)=w465) -> (created path=w464:path)  [unwired: 2 in, 2 out]
                        }
                      }
                      n137 = List Folder(path=w448) -> (folder names=w450:string[])  [unwired: 3 in, 3 out]
                      n138 = Search 1D Array(1D array=w450, element=w447) -> (index of element=w449:i32)  [unwired: 1 in]
                      n139 = Build Path(base path=w448, name or relative path=w447) -> (appended path=w446:path)
                      n140 = case shown="-1" w449 {
                        tunnel: w446 -> [w460 w462]
                        tunnel: [w460 w461] -> w439
                        frame Default {
                        }
                        frame -1 {
                          n141 = Create Folder(path (use dialog)=w462) -> (created path=w461:path)  [unwired: 2 in, 2 out]
                        }
                      }
                      n142 = Build Path(base path=w439, name or relative path=w441) -> (appended path=w440:path)
                      n143 = Open/Create/Replace File(file path (use dialog)=w440, operation (0:open)=T6."create") -> (refnum out=w458:refnum<file>, cancelled=w452:bool, error out=w451:errorcluster)  [unwired: 4 in]
                    }
                    frame 1 {
                      (unwired) "\n"
                      n144 = Concatenate Strings("Configurations" ("format string"), "\r") -> (w480:string)
                      n145 = Write to Text File(file (use dialog)=w478, text=w480, error in=w476) -> (refnum out=w475:refnum<file>, error out=w477:errorcluster)  [unwired: 1 in, 1 out]
                      n146 = for {
                        tunnel: w479 -> [w484] mode=indexing
                        shift-right: [w488] -> w473
                        shift-left: w475 -> [w488]
                        shift-right: [w487] -> w472
                        shift-left: w477 -> [w487]
                        tunnel: [w486] -> w474 mode=concatenating
                        n147 = property class="Ctl"(reference=w484) -> (reference out=w485:refnum<vi>, "ClassName"=w483:string)  [unwired: 1 in, 1 out]
                        n148 = case shown="\"Digital\"" w483 {
                          tunnel: [_ w492] -> w486
                          tunnel: w485 -> [_ w490]
                          frame Default {
                          }
                          frame "Digital" {
                            w489 = refnum<vi> refnum  # Digital
                            n149 = To More Specific Class(target class=w489, reference=w490) -> (specific class reference=w491:refnum<vi>)  [unwired: 1 in, 1 out]
                            n150 = property class="DigNum"(reference=w491) -> ("Label.Text"=w497:string, "NumText.Text"=w496:string)  [unwired: 1 in, 2 out]
                            n151 = Build Array(w497, w496) -> (w493:string[])
                            n152 = Array To Spreadsheet String(delimiter (Tab)=",", array=w493, 3:"" ("format string")) -> (spreadsheet string=w492:string)
                          }
                        }
                      }
                      n153 = Write to Text File(file (use dialog)=w473, text=w474, error in=w472) -> (refnum out=w468:refnum<file>, error out=w470:errorcluster)  [unwired: 1 in, 1 out]
                      n154 = Write to Text File(file (use dialog)=w468, text="\n", error in=w470) -> (refnum out=w467:refnum<file>, error out=w469:errorcluster)  [unwired: 1 in, 1 out]
                    }
                    frame 2 {
                      n155 = Concatenate Strings("Results" ("element"), "\r") -> (w500:string)
                      n156 = Write to Text File(file (use dialog)=w514, text=w500, error in=w513) -> (refnum out=w512:refnum<file>, error out=w508:errorcluster)  [unwired: 1 in, 1 out]
                      n157 = Array To Spreadsheet String(delimiter (Tab)=",", array=string[] ["Scope", "Channel", "Pk-Pk Ripple (V) ", "Minimum (V)", "Maximum (V)"], 3:"" ("format string")) -> (spreadsheet string=w509:string)
                      n158 = Write to Text File(file (use dialog)=w512, text=w509, error in=w508) -> (refnum out=w507:refnum<file>, error out=w506:errorcluster)  [unwired: 1 in, 1 out]
                      n159 = Write to Text File(file (use dialog)=w507, text="\n", error in=w506) -> (refnum out=w505:refnum<file>, error out=w504:errorcluster)  [unwired: 1 in, 1 out]
                    }
                    frame 3 {
                      n160 = Unbundle By Name(w520) -> ("Measurement Results.Ripple values"=w519:dbl[], "Measurement Results.Min values"=w518:dbl[], "Measurement Results.Max values"=w517:dbl[])
                      n161 = for {
                        tunnel: [w542] -> w516 mode=indexing
                        tunnel: w519 -> [w541] mode=indexing
                        tunnel: w518 -> [w540] mode=indexing
                        tunnel: w517 -> [w539] mode=indexing
                        tunnel: w521 -> [w535] mode=indexing
                        tunnel: w522 -> [w536] mode=indexing
                        n162 = Build Array(w541, w540, w539) -> (w538:dbl[])
                        n163 = Build Array(w536, w535) -> (w534:string[])
                        n164 = for {
                          tunnel: w534 -> [w545] mode=indexing
                          tunnel: [w544] -> w533 mode=indexing
                          n165 = Format Into String(format string="%s" ("initial string"), w545) -> (resulting string=w544:string)  [unwired: 2 in, 1 out]
                        }
                        n166 = for {
                          tunnel: w538 -> [w548] mode=indexing
                          tunnel: [w547] -> w537 mode=indexing
                          n167 = Format Into String(format string="%.6f" ("initial string"), w548) -> (resulting string=w547:string)  [unwired: 2 in, 1 out]
                        }
                        n168 = Build Array (concatenate)(w533, w537) -> (w542:string[])
                      }
                      n169 = Array To Spreadsheet String(delimiter (Tab)=",", array=w516, 3:"" ("format string")) -> (spreadsheet string=w528:string)
                      n170 = Write to Text File(file (use dialog)=w532, text=w528, error in=w531) -> (refnum out=w527:refnum<file>, error out=w526:errorcluster)  [unwired: 1 in, 1 out]
                      n171 = Write to Text File(file (use dialog)=w527, text="\n", error in=w526) -> (refnum out=w525:refnum<file>, error out=w524:errorcluster)  [unwired: 1 in, 1 out]
                    }
                    frame 4 {
                      n172 = Close File(refnum=w553, error in=w550) -> (error out=w551:errorcluster)  [unwired: 1 out]
                    }
                    frame 5 {
                      n173 = Get Date/Time In Seconds() -> (seconds since 1Jan1904=w560:timestamp)
                      n174 = Format Date/Time String(time format string (%c)="%Y-%m-%d %H-%M-%S", seconds (now)=w560) -> (date/time string=w559:string)  [unwired: 1 in]
                      n175 = Concatenate Strings(w559, ".png" ("string")) -> (w557:string)
                      n176 = Build Path(base path=w556, name or relative path=w557) -> (appended path=w554:path)
                      n177 = invoke on="CrosstalkGraph" class="WFGraph (strict)" method="Get Image"() -> ("image data"=w555:T14)  [unwired: 6 in, 5 out]
                      n178 = call <vilib>:"Write PNG File.vi"("image data"=w555, "path to PNG file"=w554) -> ()  [unwired: 8 in, 2 out]
                    }
                    frame Default {
                    }
                  }
                }
              }
              frame False {
              }
            }
          }
          frame "Exit", Default {
            # "Aborts and closes all the opened sessions"
            n179 = Release Queue(queue=w569, error in (no error)=w574) -> (error out=w573:errorcluster)  [unwired: 1 in, 2 out]
            n180 = case shown="No Error" w573 {
              selector: w573 -> [w580 w608]
              tunnel: [w581 w619] -> w571
              tunnel: w572 -> [w582 w618]
              tunnel: [w589 w618] -> w570
              frame No Error {
                # "Updates the status indicator on the operation performed if there is no error"
                n181 = Unbundle By Name(w582) -> ("Source out"=w588:refnum<k15>, "Source channel name"=w584:string, "Load out"=w576:refnum<k15>, "Load channel name"=w587:string, "Scopes out"=w578:refnum<k15>[])
                n182 = for {
                  shift-right: [w598] -> w579
                  shift-left: w580 -> [w599]
                  tunnel: w578 -> [w597] mode=indexing
                  n183 = call <instrlib>:"niScope Abort.vi"("instrument handle"=w597, "error in"=w599) -> ("instrument handle out"=w600:refnum<k15>, "error out"=w601:errorcluster)  [unwired: 12 in]
                  n184 = call <instrlib>:"niScope Close.vi"("instrument handle"=w600, "error in"=w601) -> ("error out"=w598:errorcluster)  [unwired: 13 in]
                }
                n185 = Empty String/Path?(string/path=w576) -> (empty?=w575:bool)
                n186 = case shown="False" w575 {
                  tunnel: w587 -> [w595 _]
                  tunnel: [w594 w596] -> w583
                  tunnel: w579 -> [w593 w596]
                  tunnel: w576 -> [w590 _]
                  frame False {
                    n187 = call <instrlib>:"niDCPower Abort With Channels.vi"("error in (no error)"=w593, "channel name"=w595, "instrument handle"=w590) -> ("error out"=w592:errorcluster, "instrument handle out"=w591:refnum<k15>)  [unwired: 7 in]
                    n188 = call <instrlib>:"niDCPower Close.vi"("error in (no error)"=w592, "instrument handle"=w591) -> ("error out"=w594:errorcluster)  [unwired: 9 in]
                  }
                  frame True {
                  }
                }
                n189 = call <instrlib>:"niDCPower Abort With Channels.vi"("error in (no error)"=w583, "channel name"=w584, "instrument handle"=w588) -> ("error out"=w586:errorcluster, "instrument handle out"=w585:refnum<k15>)  [unwired: 7 in]
                n190 = call <instrlib>:"niDCPower Close.vi"("error in (no error)"=w586, "instrument handle"=w585) -> ("error out"=w581:errorcluster)  [unwired: 9 in]
                n191 = Bundle By Name(cluster=w582, "Measurement Results.Status"="The measurement is performed successfully" ("message")) -> (w589:T3)
              }
              frame Error {
                # "Resets the device with default values whenever there is an error"
                n192 = Unbundle By Name(w618) -> ("Source out"=w613:refnum<k15>, "Source channel name"=w611:string, "Load out"=w610:refnum<k15>, "Load channel name"=w609:string, "Scopes out"=w606:refnum<k15>[])
                n193 = for {
                  shift-right: [w621] -> w607
                  shift-left: w608 -> [w622]
                  tunnel: w606 -> [w620] mode=indexing
                  n194 = call <instrlib>:"niScope Abort.vi"("instrument handle"=w620, "error in"=w622) -> ("instrument handle out"=w626:refnum<k15>, "error out"=w625:errorcluster)  [unwired: 12 in]
                  n195 = call <instrlib>:"niScope Reset.vi"("instrument handle"=w626, "error in"=w625) -> ("instrument handle out"=w624:refnum<k15>, "error out"=w623:errorcluster)  [unwired: 12 in]
                  n196 = call <instrlib>:"niScope Close.vi"("instrument handle"=w624, "error in"=w623) -> ("error out"=w621:errorcluster)  [unwired: 13 in]
                }
                n197 = call <instrlib>:"niDCPower Abort With Channels.vi"("error in (no error)"=w607, "channel name"=w609, "instrument handle"=w610) -> ("error out"=w603:errorcluster, "instrument handle out"=w602:refnum<k15>)  [unwired: 7 in]
                n198 = call <instrlib>:"niDCPower Reset With Channels.vi"("error in (no error)"=w603, "channel name"=w609, "instrument handle"=w602) -> ("error out"=w604:errorcluster, "instrument handle out"=w605:refnum<k15>)  [unwired: 7 in]
                n199 = call <instrlib>:"niDCPower Close.vi"("error in (no error)"=w604, "instrument handle"=w605) -> ("error out"=w612:errorcluster)  [unwired: 9 out]
                n200 = call <instrlib>:"niDCPower Abort With Channels.vi"("error in (no error)"=w612, "channel name"=w611, "instrument handle"=w613) -> ("error out"=w614:errorcluster, "instrument handle out"=w615:refnum<k15>)  [unwired: 7 in]
                n201 = call <instrlib>:"niDCPower Reset With Channels.vi"("error in (no error)"=w614, "channel name"=w611, "instrument handle"=w615) -> ("error out"=w617:errorcluster, "instrument handle out"=w616:refnum<k15>)  [unwired: 7 in]
                n202 = call <instrlib>:"niDCPower Close.vi"("error in (no error)"=w617, "instrument handle"=w616) -> ("error out"=w619:errorcluster)  [unwired: 9 out]
              }
            }
          }
        }
      }
    }
    frame "Power off the DUT" {
      # "Stops generation on the output channel and resets the channels to default values"
      n203 = Unbundle By Name(w656) -> ("Source resource name"=w658:string, "Load resource name"=w660:string)
      n204 = call <instrlib>:"niDCPower Initialize With Independent Channels.vi"("error in (no error)"=w666, "resource name"=w660) -> ("error out"=w642:errorcluster, "instrument handle out"=w641:refnum<k15>)  [unwired: 8 in]
      n205 = call-poly <instrlib>:"niDCPower Get Channel Name (Poly).vi"("error in (no error)"=w642, "index"="0", "instrument handle"=w641) -> ("error out"=w646:errorcluster, "name"=w643:string, "instrument handle out"=w644:refnum<k15>)  [unwired: 6 in]
      n206 = call <instrlib>:"niDCPower Configure Output Enabled.vi"("error in (no error)"=w646, "output enabled"=FALSE, "channel name"=w643, "instrument handle"=w644) -> ("error out"=w651:errorcluster, "instrument handle out"=w650:refnum<k15>)  [unwired: 6 in]
      n207 = call <instrlib>:"niDCPower Reset With Channels.vi"("error in (no error)"=w651, "channel name"=w643, "instrument handle"=w650) -> ("error out"=w647:errorcluster, "instrument handle out"=w648:refnum<k15>)  [unwired: 7 in]
      n208 = call <instrlib>:"niDCPower Close.vi"("error in (no error)"=w647, "instrument handle"=w648) -> ("error out"=w663:errorcluster)  [unwired: 9 out]
      n209 = call <instrlib>:"niDCPower Initialize With Independent Channels.vi"("error in (no error)"=w663, "resource name"=w658) -> ("error out"=w659:errorcluster, "instrument handle out"=w657:refnum<k15>)  [unwired: 8 in]
      n210 = call-poly <instrlib>:"niDCPower Get Channel Name (Poly).vi"("error in (no error)"=w659, "index"="0", "instrument handle"=w657) -> ("error out"=w662:errorcluster, "name"=w661:string, "instrument handle out"=w664:refnum<k15>)  [unwired: 6 in]
      n211 = call <instrlib>:"niDCPower Reset With Channels.vi"("error in (no error)"=w662, "channel name"=w661, "instrument handle"=w664) -> ("error out"=w669:errorcluster, "instrument handle out"=w668:refnum<k15>)  [unwired: 7 in]
      n212 = call <instrlib>:"niDCPower Close.vi"("error in (no error)"=w669, "instrument handle"=w668) -> ("error out"=w667:errorcluster)  [unwired: 9 out]
      n213 = Bundle By Name(cluster=w654, "Measurement Results.Status"="The DUT is powered OFF") -> (w653:T3)
    }
  }
  "error out" <- w4
  "measure call context out" <- w5
  n214 = Unbundle By Name(w2) -> ("Measurement Results"=→"measurement results":T1)
